vi "Map Attributes.vi"(4 "attributes":map{string, variant}(c390), 5 "record":T1, 8 "error in":errorcluster) -> (0 "error out":errorcluster, 1 "counts out":map{string, u64}(c390), 2 "attributes out":map{string, variant}(c390), 3 "record out":T1)   [LabVIEW 2026]
doc: "Pass a map and a cluster holding a map through."
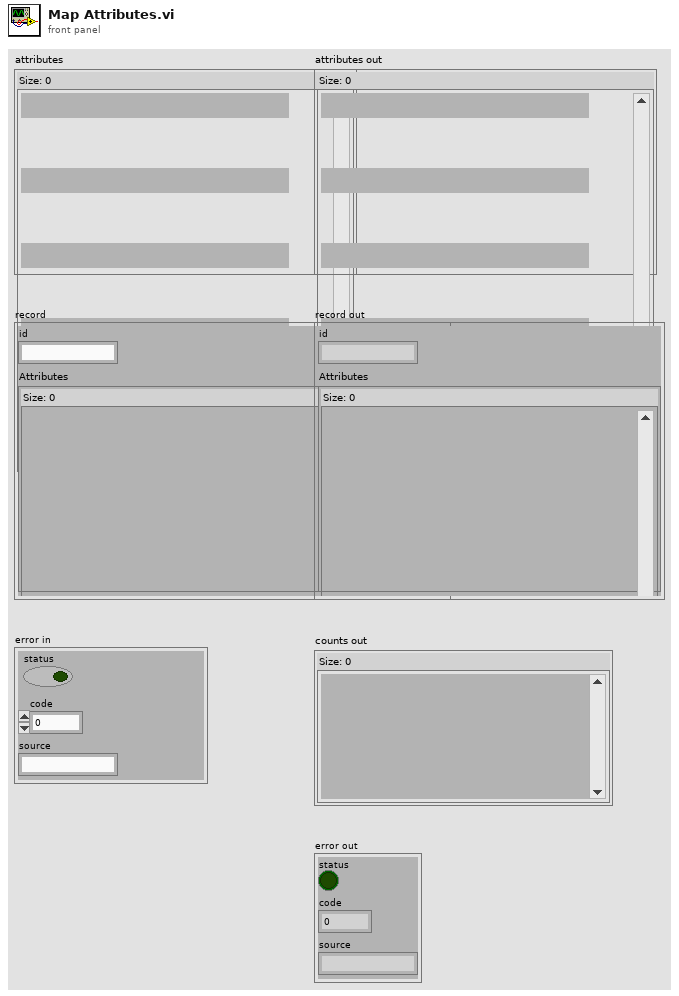
[diagram p1: front panel]
types:
  T1 = cluster{"id":string, "Attributes":map{string, variant}}
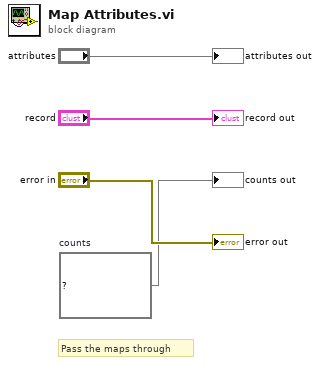
[diagram p0: block diagram]
diagram:
  w3 = map{string, u64} {}  # counts
  # "Pass the maps through"
  "attributes out" <- "attributes"
  "record out" <- "record"
  "counts out" <- w3
  "error out" <- "error in"
